vi "Filter Wheel Messenger.vi"(0 "FW Notifier":string, 2 "Actions":T1, 11 "Set Position":u8, 13 "Exit While Busy?":bool) -> (4 "FW Notifier (Dup)":string, 8 "Num Positions":u8, 15 "Current Position":u8)   [LabVIEW 2016]
uses:
  FW Type Defs/FW Actions.ctl
  FW Type Defs/FW Notifier Type.ctl
panel:
  out "Error":errorcluster
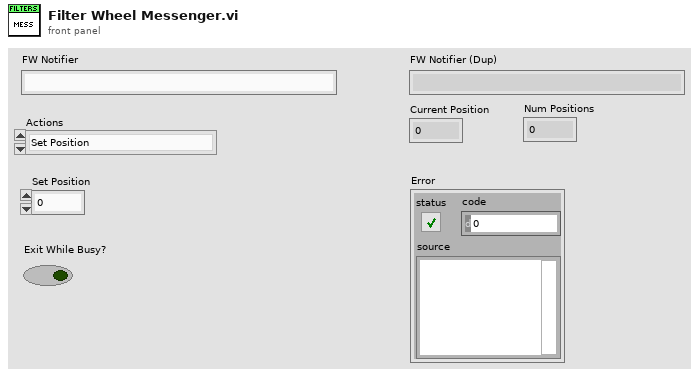
[diagram p1: front panel]
types:
  T1 = typedef "FW Actions.ctl" = enum16{"Set Position", "Get Position", "Get Num Positions", "Set Speed", "Quit"}
  T2 = typedef "FW Notifier Type.ctl" = cluster{"Actions":T1, "Set Position":u8, "Actual Position":u8, "Speed":dbl, "Num Positions":u8, "Received":bool}
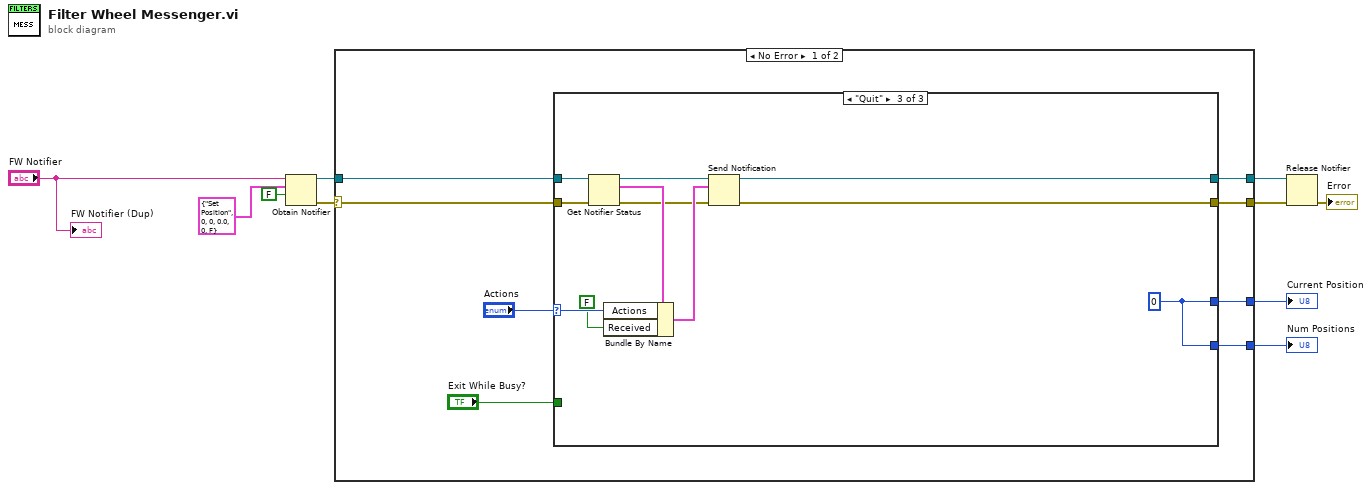
[diagram p0: block diagram]
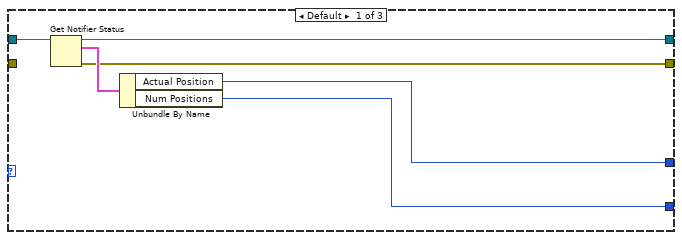
[diagram p2: hidden frame]
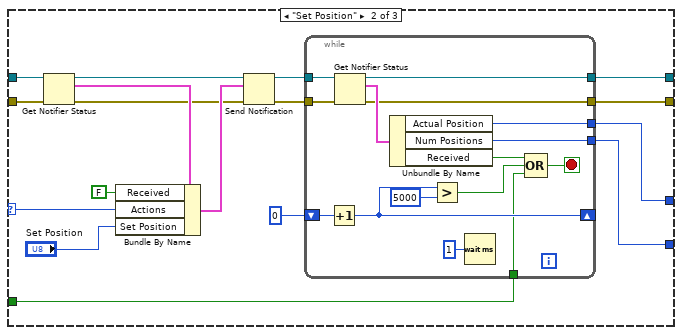
[diagram p3: hidden frame]
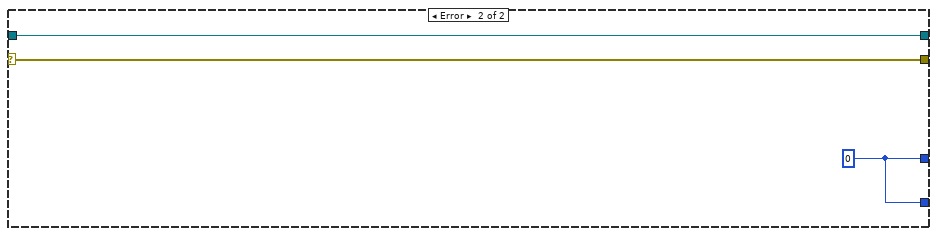
[diagram p4: hidden frame]
diagram:
  n1 = Obtain Notifier(name (unnamed)="FW Notifier", notification data type=T2 {"Actions"=enum."Set Position", "Set Position"=0, "Actual Position"=0, "Speed"=0.0, "Num Positions"=0, "Received"=FALSE} ("FW102C Note Type"), create if not found? (T)=FALSE) -> (notifier out=w7:refnum<notifier>, error out=w8:errorcluster)  [unwired: 1 in, 1 out]
  n2 = case shown="No Error" w8 {
    selector: w8 -> [w12 w69]
    tunnel: w7 -> [w13 w70]
    tunnel: [w16 w68] -> w6
    tunnel: [w15 w70] -> w4
    tunnel: [w14 w69] -> w3
    tunnel: [w11 w68] -> w1
    frame No Error {
      n3 = case shown="\"Quit\"" "Actions" {
        selector: "Actions" -> [_ w38 w64]
        tunnel: w13 -> [w24 w41 w67]
        tunnel: [w22 w26 w57] -> w16
        tunnel: "Exit While Busy?" -> [_ w33 _]
        tunnel: w12 -> [_ w31 w62]
        tunnel: [w21 w32 w60] -> w15
        tunnel: [w20 w28 w59] -> w14
        tunnel: [w19 w25 w57] -> w11
        frame Default {
          n4 = Get Notifier Status(notifier=w24) -> (notifier out=w21:refnum<notifier>, current notification=w23:T2, error out=w20:errorcluster)  [unwired: 1 in, 2 out]
          n5 = Unbundle By Name(w23) -> ("Actual Position"=w22:u8, "Num Positions"=w19:u8)
        }
        frame "Set Position" {
          n6 = Get Notifier Status(notifier=w41, error in (no error)=w31) -> (notifier out=w40:refnum<notifier>, current notification=w39:T2, error out=w30:errorcluster)  [unwired: 2 out]
          n7 = Bundle By Name(cluster=w39, "Received"=FALSE, "Actions"=w38, "Set Position"="Set Position") -> (w36:T2)
          n8 = Send Notification(notification=w36, notifier=w40, error in (no error)=w30) -> (notifier out=w35:refnum<notifier>, error out=w29:errorcluster)
          n9 = while {
            tunnel: w35 -> [w56]
            shift-right: [w51] -> _
            shift-left: u16 0 -> [w52]
            tunnel: [w42] -> w25
            tunnel: w33 -> [w48]
            tunnel: [w46] -> w32
            tunnel: w29 -> [w45]
            tunnel: [w44] -> w28
            tunnel: [w43] -> w26
            stop <- w53 stop-if-true
            n10 = Increment(x=w52) -> (x+1=w51:u16)
            n11 = Get Notifier Status(notifier=w56, error in (no error)=w45) -> (notifier out=w46:refnum<notifier>, current notification=w55:T2, error out=w44:errorcluster)  [unwired: 2 out]
            n12 = Unbundle By Name(w55) -> ("Actual Position"=w43:u8, "Num Positions"=w42:u8, "Received"=w54:bool)
            n13 = Greater?(x=w51, y=u16 5000) -> (0:w49:bool)
            n14 = Wait (ms)(milliseconds to wait=u32 1) -> ()  [unwired: 1 out]
            n15 = Compound Arithmetic op=OR(w54, w49, w48) -> (w53:bool)
          }
        }
        frame "Quit" {
          w57 = u8 0 ("Actual Position")
          n16 = Get Notifier Status(notifier=w67, error in (no error)=w62) -> (notifier out=w66:refnum<notifier>, current notification=w65:T2, error out=w61:errorcluster)  [unwired: 2 out]
          n17 = Bundle By Name(cluster=w65, "Actions"=w64, "Received"=FALSE) -> (w63:T2)
          n18 = Send Notification(notification=w63, notifier=w66, error in (no error)=w61) -> (notifier out=w60:refnum<notifier>, error out=w59:errorcluster)
        }
      }
    }
    frame Error {
      w68 = u8 0 ("Actual Position")
    }
  }
  "Current Position" <- w6
  "Num Positions" <- w1
  n19 = Release Notifier(notifier=w4, error in (no error)=w3) -> (error out=→"Error":errorcluster)  [unwired: 1 in, 2 out]
  "FW Notifier (Dup)" <- "FW Notifier"
